vi "Range-check-csm-works.vi"(7 "UUID":string="Range check") -> ()   [LabVIEW 2018]
uses:
  <userlib>/_NEVSTOP/Communicable State Machine(CSM)/_Support/Typedef/_CSM_MODE.ctl
  API.ctl
  c61bc4df-35aa-4b4d-b5cf-ea0051ca23be.vi
  0e4ee468-faba-4892-866f-7e2dcb46ee8c.vi
  <userlib>/_NEVSTOP/Communicable State Machine(CSM)/AdvanceAPI/CSM - Revert Arguments-Safe String.vi
  <userlib>/_NEVSTOP/Communicable State Machine(CSM)/_Shared/Trim Single-line Text.vi
  <userlib>/_NEVSTOP/Communicable State Machine(CSM)/AdvanceAPI/CSM - Make String Arguments Safe.vi
  <userlib>/_NEVSTOP/Communicable State Machine(CSM)/AdvanceAPI/CSM - Break Down Multiple States String.vi
  <userlib>/_NEVSTOP/Communicable State Machine(CSM)/AdvanceAPI/CSM - Compact Multiple States.vi
  <userlib>/_NEVSTOP/Communicable State Machine(CSM)/AdvanceAPI/CSM - Keywords.vi
  <userlib>/_NEVSTOP/Communicable State Machine(CSM)/addons/API-String-Arugments-Support/_Support/Convert API String Arguments to Data(variant).vi
  <userlib>/_NEVSTOP/Communicable State Machine(CSM)/addons/API-String-Arugments-Support/_Support/Data To API String Arguments.vi
  <userlib>/_NEVSTOP/Communicable State Machine(CSM)/_Polymophic/Build Asynchronous Message with Arguments.vi
  <vilib>/regexp/Match Regular Expression.xnode
  <userlib>/_NEVSTOP/Communicable State Machine(CSM)/Communicable State Machine.lvlib
  <userlib>/_NEVSTOP/Communicable State Machine(CSM)/addons/Loop-Support/CSM Loop Support.lvlib
panel:
  out "输出簇":T2(array[cluster])
  out "Error Occurred":errorcluster
  out "State History":string
  # "借用CSM的works模式\n需要Timer CSM Works库---\n注意，由于退出机制的设置，本VI无论有多少个，一旦一个退出，其附带的所有的Timer-works都会退出\n没有办法，我并不能知道那个正在使用中\\\n本VI的API只能使用异步消息\n结果的返回是通过广播，所以需要你去注册对应广播"
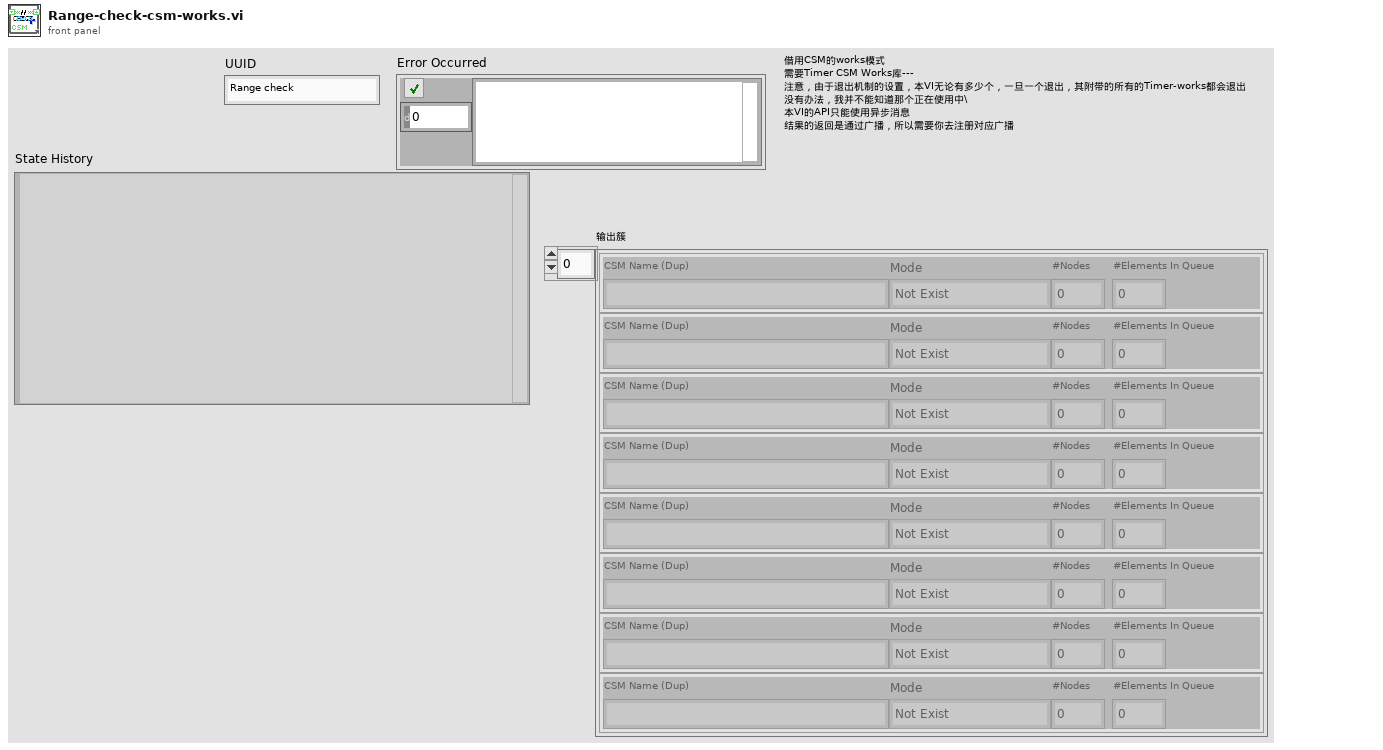
[diagram p1: front panel]
types:
  T1 = typedef "Communicable State Machine.lvlib/_CSM_MODE.ctl" = enum16{"Not Exist", "Stand Alone", "CSM", "Worker", "Worker Agent", "Chain Node", "Chain"}
  T2 = cluster{"CSM Name (Dup)":string, "Mode":T1, "#Nodes":i32, "#Elements In Queue":i32}[]
  T3 = enum32{"Invalid", "Standard", "Closed", "Hidden", "Minimized", "Maximized"}
  T4 = enum32{"invalid app kind", "Development System", "Run Time System", "Student Edition", "Embedded LabVIEW", "Evaluation", "Custom"}
  T5 = typedef "Communicable State Machine.lvlib/_CSM_Response Source Message.ctl" = cluster{"‘State":string, "’Arguments":string, "’Error":errorcluster}
  T6 = cluster{"Current VI Reference":refnum<vi>, "Close Panel on Exit?":bool}
  T7 = typedef "API.ctl" = cluster{"设定值上限":dbl, "设定值下限":dbl, "设定时间ms":u32, "超时时间ms":u32}
  T8 = cluster{"Core":cluster{"Current VI Reference":refnum<vi>, "Close Panel on Exit?":bool}, "Timing Parameters":T7, "Start":u32, "Esplase time":u32, "Success？":bool, "Time out？":bool, "Source":string, "ALL time":u32, "ALL Start":u32, "My name":string}
  T9 = cluster{"设定值上限":dbl, "设定值下限":dbl, "设定时间ms":dbl, "超时时间ms":dbl}
  T10 = cluster{"CSM Name (Dup)":string, "Mode":T1, "#Nodes":i32, "#Elements In Queue":i32}
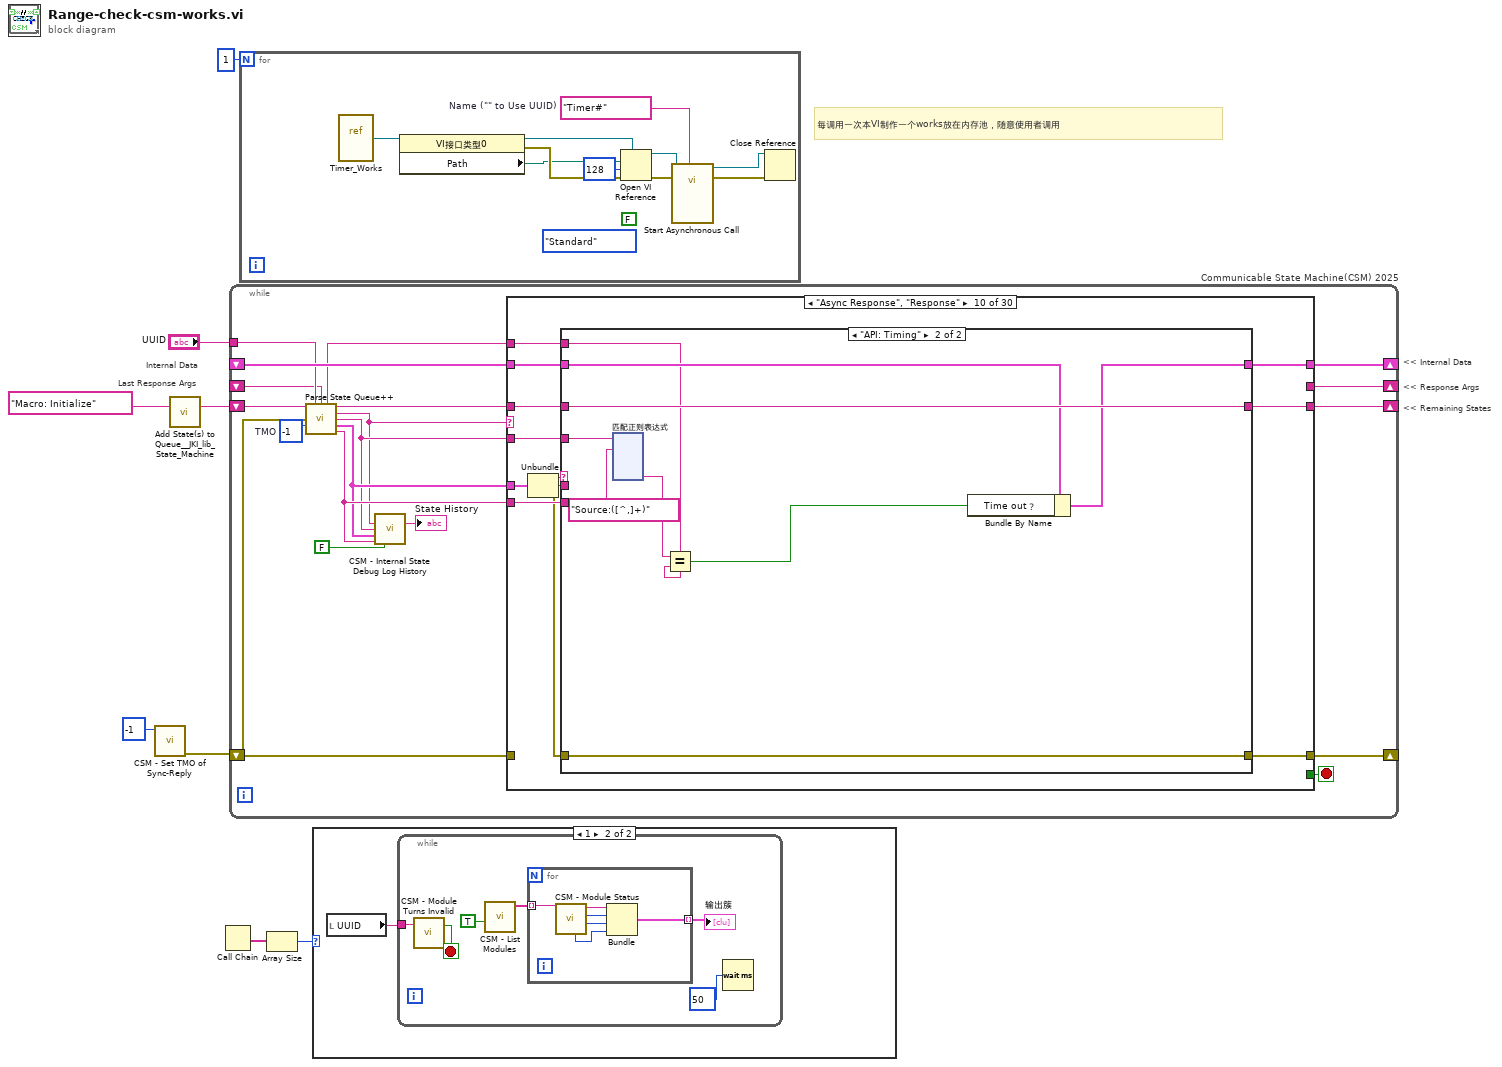
[diagram p0: block diagram]
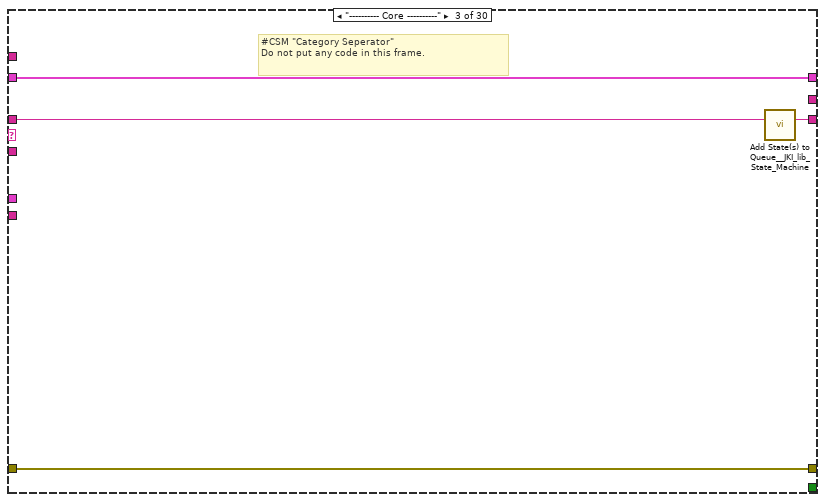
[diagram p5: hidden frame]
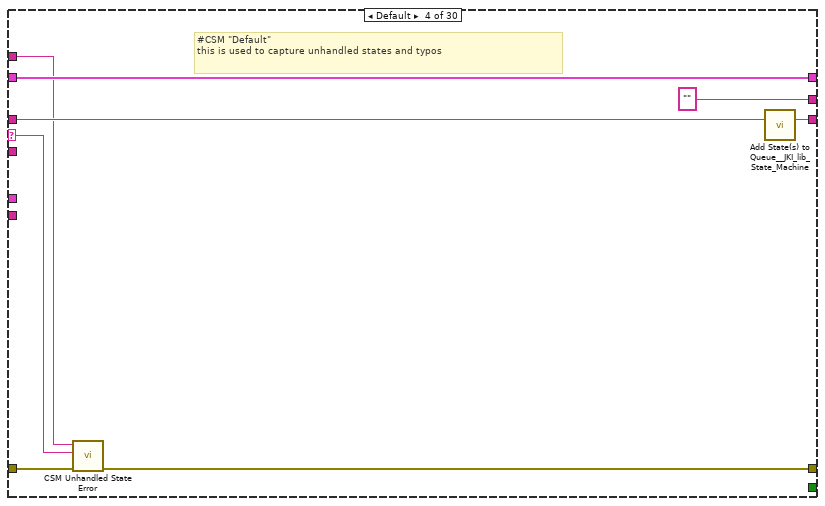
[diagram p6: hidden frame]
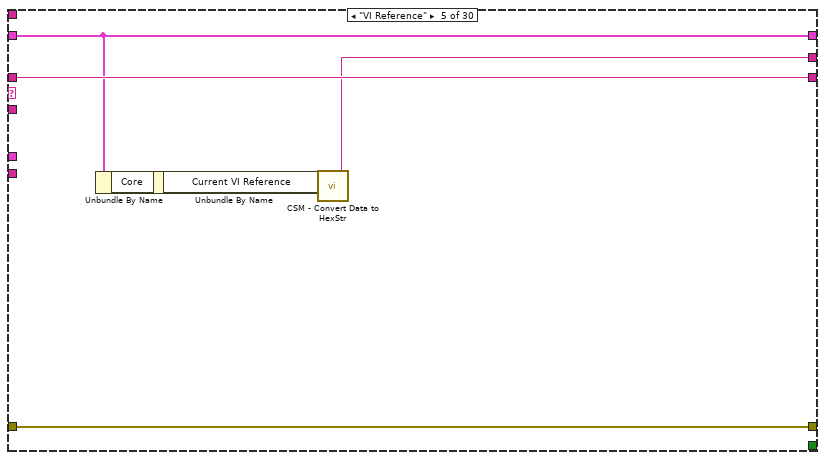
[diagram p7: hidden frame]
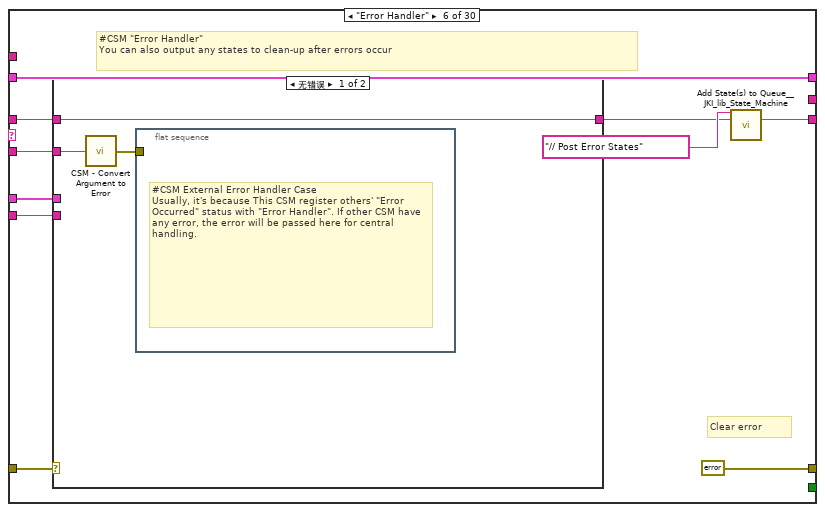
[diagram p8: hidden frame]
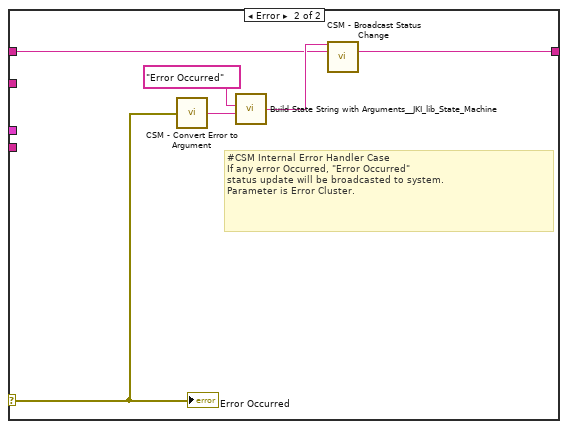
[diagram p9: hidden frame]
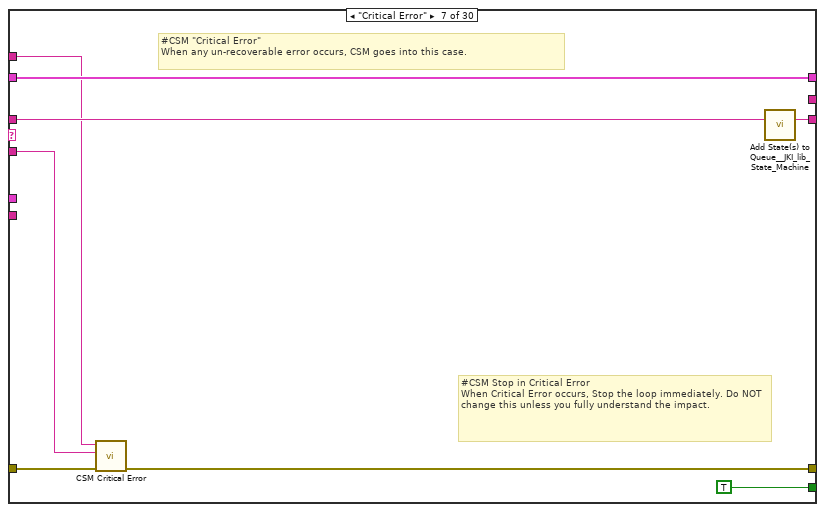
[diagram p10: hidden frame]
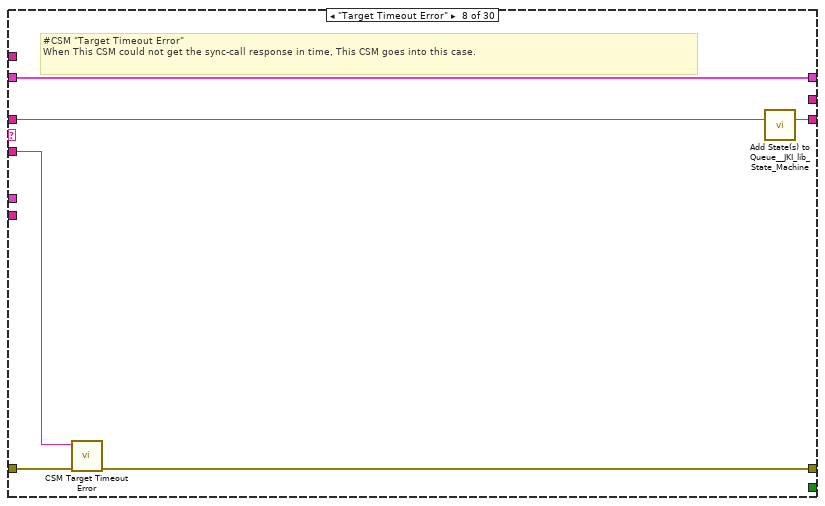
[diagram p11: hidden frame]
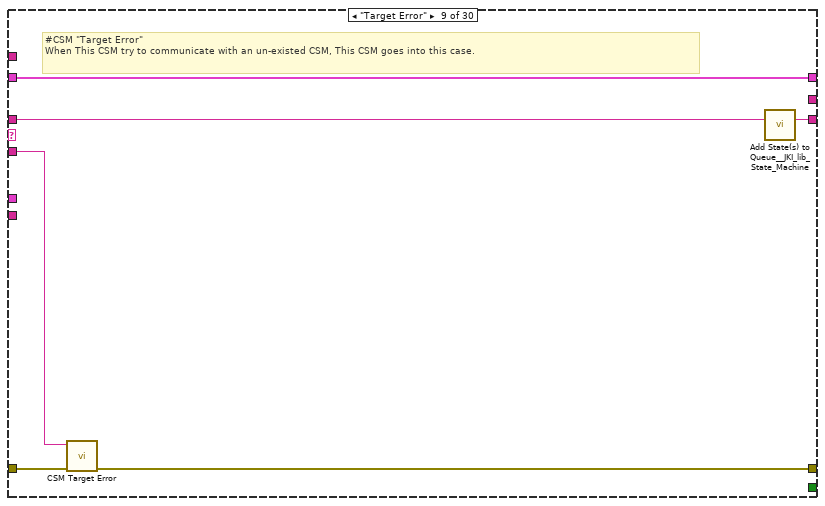
[diagram p12: hidden frame]
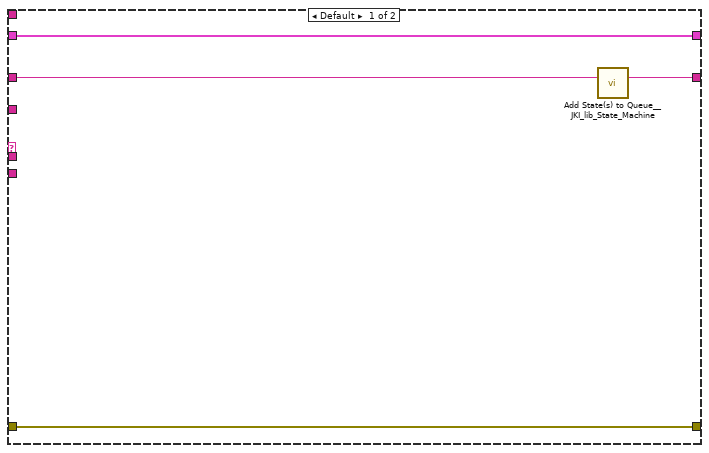
[diagram p13: hidden frame]
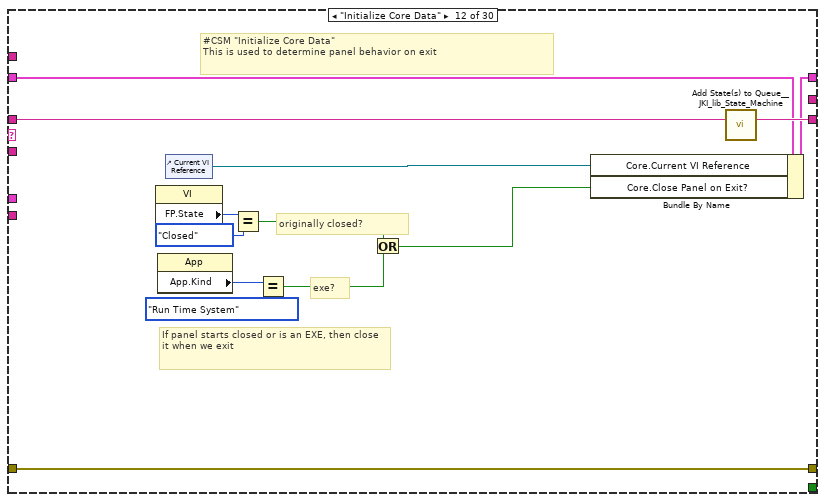
[diagram p15: hidden frame]
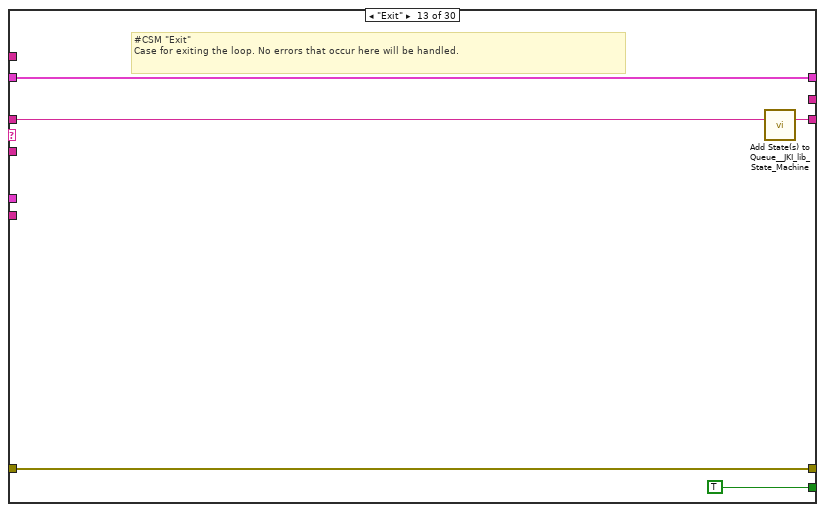
[diagram p16: hidden frame]
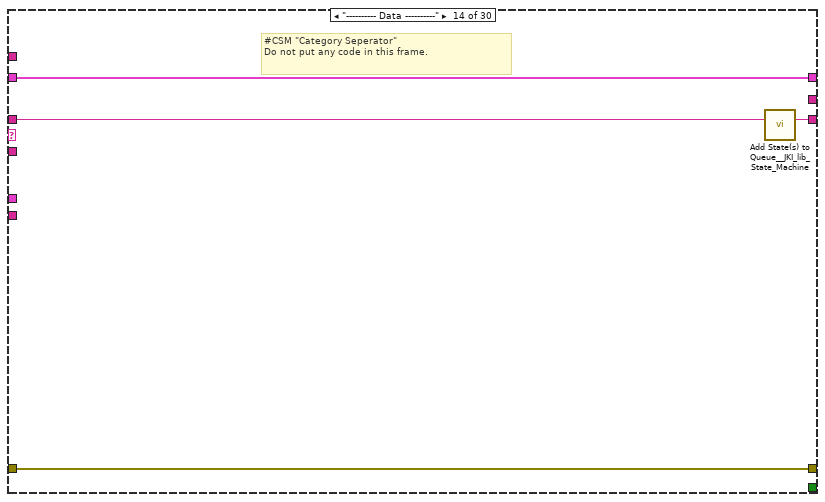
[diagram p17: hidden frame]
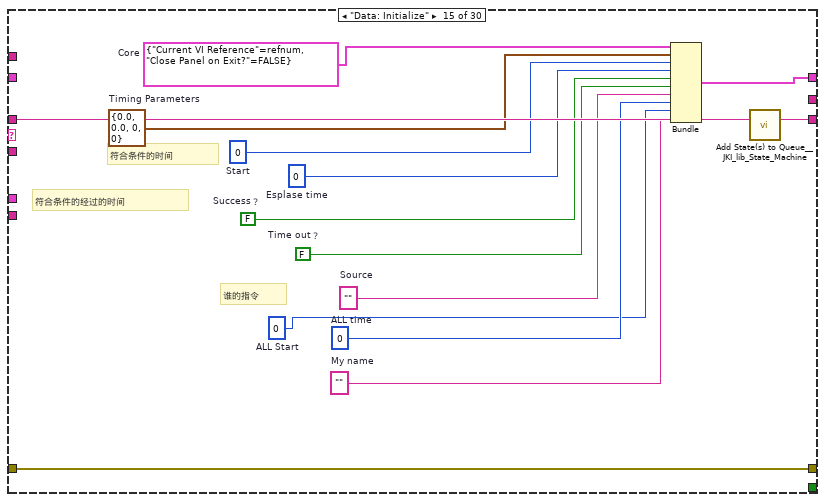
[diagram p18: hidden frame]
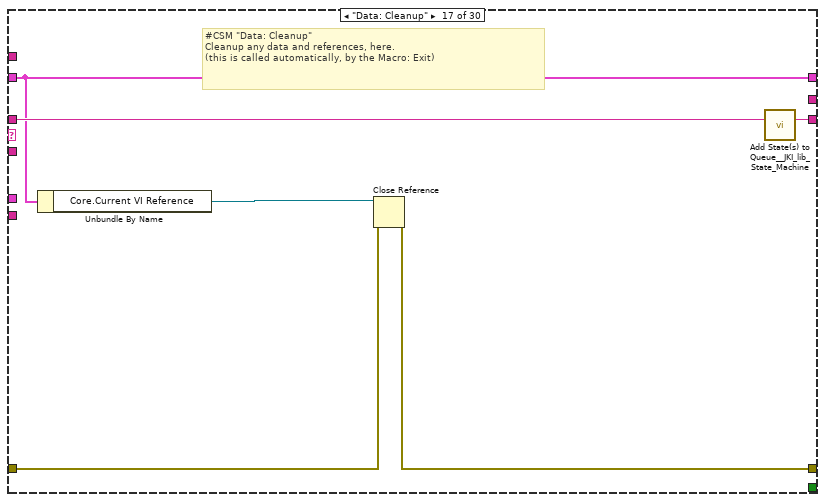
[diagram p20: hidden frame]
diagram:
  # "每调用一次本VI制作一个works放在内存池，随意使用者调用"
  # "Last Response Args"
  # "Internal Data"
  # "<< Internal Data"
  # "<< Response Args"
  # "<< Remaining States"
  n1 = call <userlib>:"CSM - Set TMO of Sync-Reply.vi"("TMO For Sync-Rep (ms) In"=-1) -> ("error out"=w3:errorcluster)  [unwired: 9 in, 1 out]
  n2 = call <vilib>:"Add State(s) to Queue__JKI_lib_State_Machine.vi"("State(s) in (\"\")"="Macro: Initialize" ("Init State(\"Macro: Initialize\")")) -> ("States Out"=w6:string)  [unwired: 14 in]
  n3 = Call Chain() -> (call chain=w1:string[])
  n4 = while "Communicable State Machine(CSM) 2025" {
    shift-right: [w22] -> _
    shift-left: _ -> [w21]
    shift-right: [w25] -> _
    shift-left: w3 -> [w11]
    shift-right: [w24] -> _
    shift-left: w6 -> [w26]
    tunnel: "UUID" -> [w18]
    shift-right: [w19] -> _
    shift-left: _ -> [w13]
    stop <- w23 stop-if-true
    w20 = -1  # TMO
    n5 = call <userlib>:"Parse State Queue++.vi"("State Queue"=w26, "Name (\"\" to Use UUID)"=w18, "Response Arguments"=w13, "Previous Error"=w11, "Dequeue (1 ms)"=w20) -> ("Name Used"=w12:string, "Remaining States"=w27:string, "Current State"=w14:string, "Arguments"=w15:string, "Additional Information"=w16:T5, "Source CSM"=w17:string)  [unwired: 5 in]
    n6 = call <userlib>:"CSM - Internal State Debug Log History.vi"("State"=w14, "Arguments (\"\")"=w15, ">> Response Source Message >>"=w16, "Source (\"\")"=w17, "Enable Periodic State Filter? (T)"=FALSE) -> ("Debug Log"=→"State History":string)  [unwired: 10 in]
    n7 = case shown="\"Async Response\", \"Response\"" w14 {
      selector: w14 -> [_ _ _ w41 _ _ _ _ _ _ _ _ _ _ _ _ _ _ _ _ _ _ _ _ _ _ _ _ w386 _]
      tunnel: w27 -> [w29 w33 w37 w45 w50 w55 w78 w84 w90 w101 w234 w247 w252 w256 w270 w273 w279 w283 w288 w294 w302 w305 w308 w320 w329 w338 w355 w378 w387 w393]
      tunnel: w15 -> [_ _ _ _ _ w54 w74 w81 w87 w96 _ _ _ _ _ _ _ _ _ _ _ _ w315 _ _ _ _ _ _ _]
      tunnel: w21 -> [w30 w32 w35 w43 w49 w60 w76 w82 w88 w92 w233 w241 w250 w254 _ w272 w274 w281 w286 w292 w300 w304 w316 w318 w327 w331 w354 w374 w385 w391]
      tunnel: [w28 w31 w34 w38 w51 errorcluster {"status"=FALSE, "code"=0, "source"=""} ("error out") w71 w79 w85 w102 w232 w235 w248 w253 w266 w271 w275 w280 w284 w290 w297 w303 w313 w317 w326 w336 w357 w376 w388 w390] -> w25
      tunnel: w11 -> [w28 w31 w34 w39 w51 w58 w72 w80 w86 _ w232 w235 w248 w253 w266 w271 w276 w280 w284 w290 w297 w303 w312 w317 w326 w336 w357 w376 w388 w390]
      tunnel: [w29 w33 w36 w44 w50 w56 w77 w83 w89 w100 w234 w246 w251 w255 w269 w273 w278 w282 w287 w293 w301 w305 w309 w319 w328 w337 w356 w377 w389 w392] -> w24
      tunnel: [_ _ _ _ _ _ TRUE _ _ _ _ _ TRUE _ _ _ _ _ _ _ _ _ _ _ _ _ _ _ _ _] -> w23
      tunnel: [w30 w32 w35 w43 w49 w60 w76 w82 w88 w99 w233 w245 w250 w254 w268 w272 w274 w281 w286 w292 w300 w304 w311 w318 w325 w331 w351 w374 w385 w391] -> w22
      tunnel: w17 -> [_ _ _ _ _ w53 _ _ _ w97 _ _ _ _ _ _ _ _ _ _ _ _ w306 _ _ _ _ _ _ _]
      tunnel: w16 -> [_ _ _ _ _ w52 _ _ _ w98 _ _ _ _ _ _ _ _ _ _ _ _ _ _ _ _ _ _ _ _]
      tunnel: [_ _ _ "" w46 _ _ _ _ _ _ _ _ _ _ _ _ _ _ _ _ _ _ _ _ _ _ _ _ _] -> w19
      tunnel: w12 -> [_ _ _ w40 _ _ w73 _ _ w91 _ _ _ _ _ _ _ _ _ _ _ _ _ _ _ _ _ _ _ _]
      frame "", "Idle" {
      }
      frame "CSM Documentation" {
      }
      frame "---------- Core ----------" {
        # "#CSM \"Category Seperator\"\nDo not put any code in this frame."
        n8 = call <vilib>:"Add State(s) to Queue__JKI_lib_State_Machine.vi"("State(s) in (\"\")"=w37) -> ("States Out"=w36:string)  [unwired: 14 in]
      }
      frame Default {
        # "#CSM \"Default\"\nthis is used to capture unhandled states and typos"
        n9 = call <userlib>:"CSM Unhandled State Error.vi"("error in (no error)"=w39, "Undefined State"=w41, "CSM Name"=w40) -> ("error out"=w38:errorcluster)  [unwired: 8 in]
        n10 = call <vilib>:"Add State(s) to Queue__JKI_lib_State_Machine.vi"("State(s) in (\"\")"=w45) -> ("States Out"=w44:string)  [unwired: 14 in]
      }
      frame "VI Reference" {
        n11 = Unbundle By Name(w49) -> ("Core"=w48:T6)
        n12 = Unbundle By Name(w48) -> ("Current VI Reference"=w47:refnum<vi>)
        n13 = call <userlib>:"CSM - Convert Data to HexStr.vi"("Variant"=w47) -> ("HEX String (0-9,A-F)"=w46:string)  [unwired: 8 in]
      }
      frame "Error Handler" {
        # "#CSM \"Error Handler\"\nYou can also output any states to clean-up after errors occur"
        # "Clear error"
        n14 = case shown="无错误" w58 {
          selector: w58 -> [_ w65]
          tunnel: [w64 w67] -> w57
          tunnel: w55 -> [w64 w66]
          tunnel: w54 -> [w63 _]
          tunnel: w53 -> [_ _]
          tunnel: w52 -> [_ _]
          frame No Error {
            n15 = call <userlib>:"CSM - Convert Argument to Error.vi"("Argument"=w63) -> ("Error"=w62:errorcluster)  [unwired: 4 in]
            n16 = flat-sequence {
              tunnel: w62 -> [_]
              frame #0 {
                # "#CSM External Error Handler Case\nUsually, it's because This CSM register others' \"Error Occurred\" status with \"Error Handler\". If other CSM have any error, the error will be passed here for central handling."
              }
            }
          }
          frame Error {
            # "#CSM Internal Error Handler Case \nIf any error Occurred, \"Error Occurred\" \nstatus update will be broadcasted to system.\nParameter is Error Cluster."
            n17 = call <userlib>:"CSM - Convert Error to Argument.vi"("Error"=w65) -> ("Argument"=w69:string)  [unwired: 4 in]
            n18 = call <vilib>:"Build State String with Arguments__JKI_lib_State_Machine.vi"("Arguments (\"\")"=w69, "State"="Error Occurred" ("Status with Arguments")) -> ("State with Arguments"=w68:string)  [unwired: 4 in]
            n19 = call <userlib>:"CSM - Broadcast Status Change.vi"("Status With Arguments"=w68, "State Queue"=w66) -> ("Remaining States"=w67:string)  [unwired: 13 in]
            "Error Occurred" <- w65
          }
        }
        n20 = call <vilib>:"Add State(s) to Queue__JKI_lib_State_Machine.vi"("State(s) in Front (\"\")"="// Post Error States", "State(s) in (\"\")"=w57) -> ("States Out"=w56:string)  [unwired: 13 in]
      }
      frame "Critical Error" {
        # "#CSM \"Critical Error\"\nWhen any un-recoverable error occurs, CSM goes into this case."
        # "#CSM Stop in Critical Error\nWhen Critical Error occurs, Stop the loop immediately. Do NOT change this unless you fully understand the impact."
        n21 = call <userlib>:"CSM Critical Error.vi"("error in (no error)"=w72, "Arugments (As Reason)"=w74, "CSM Name"=w73) -> ("error out"=w71:errorcluster)  [unwired: 8 in]
        n22 = call <vilib>:"Add State(s) to Queue__JKI_lib_State_Machine.vi"("State(s) in (\"\")"=w78) -> ("States Out"=w77:string)  [unwired: 14 in]
      }
      frame "Target Timeout Error" {
        # "#CSM \"Target Timeout Error\"\nWhen This CSM could not get the sync-call response in time, This CSM goes into this case."
        n23 = call <userlib>:"CSM Target Timeout Error.vi"("error in (no error)"=w80, "Arguments (As CSM Name)"=w81) -> ("error out"=w79:errorcluster)  [unwired: 9 in]
        n24 = call <vilib>:"Add State(s) to Queue__JKI_lib_State_Machine.vi"("State(s) in (\"\")"=w84) -> ("States Out"=w83:string)  [unwired: 14 in]
      }
      frame "Target Error" {
        # "#CSM \"Target Error\"\nWhen This CSM try to communicate with an un-existed CSM, This CSM goes into this case."
        n25 = call <userlib>:"CSM Target Error.vi"("error in (no error)"=w86, "Arguments (As CSM Name)"=w87) -> ("error out"=w85:errorcluster)  [unwired: 9 in]
        n26 = call <vilib>:"Add State(s) to Queue__JKI_lib_State_Machine.vi"("State(s) in (\"\")"=w90) -> ("States Out"=w89:string)  [unwired: 14 in]
      }
      frame "Async Response", "Response" {
        n27 = Unbundle(w98) -> ("‘State"=w95:string, "’Arguments"=w94:string, "’Error"=w93:errorcluster)
        n28 = case shown="\"API: Timing\"" w95 {
          tunnel: [w104 w115] -> w100
          tunnel: w101 -> [w105 w115]
          tunnel: [w103 w110] -> w99
          tunnel: [w106 w114] -> w102
          tunnel: w93 -> [w106 w114]
          tunnel: w97 -> [_ _]
          tunnel: w96 -> [_ w113]
          tunnel: w94 -> [_ _]
          tunnel: w92 -> [w103 w108]
          tunnel: w91 -> [_ w107]
          frame Default {
            n29 = call <vilib>:"Add State(s) to Queue__JKI_lib_State_Machine.vi"("State(s) in (\"\")"=w105) -> ("States Out"=w104:string)  [unwired: 14 in]
          }
          frame "API: Timing" {
            n30 = xnode "匹配正则表达式"("输入字符串"=w113, "正则表达式"="Source:([^,]+)") -> ("子匹配 1"=w111:string)  [unwired: 4 in, 5 out]
            n31 = Equal?(x=w111, y=w107) -> (x = y?=w109:bool)
            n32 = Bundle By Name(cluster=w108, "Time out？"=w109) -> (w110:T8)
          }
        }
      }
      frame "Async Message Posted" {
        # "#CSM \"Async Message Posted\"\nAfter Async Message is posted (-> or ->| ), CSM goes to this state for post-action.\nYou can use Argument - State to tell which Async Message is called."
      }
      frame "Initialize Core Data" {
        # "#CSM \"Initialize Core Data\"\nThis is used to determine panel behavior on exit"
        # "originally closed?"
        # "exe?"
        # "If panel starts closed or is an EXE, then close it when we exit"
        n33 = property class="VI"() -> ("FP.State"=w238:T3)  [unwired: 2 in, 2 out]
        n34 = property class="App"() -> ("App.Kind"=w244:T4)  [unwired: 2 in, 2 out]
        n35 = control-ref of="Current VI Reference"() -> (w239:refnum<vi>)
        n36 = Equal?(x=w238, y=T3."Closed" ("Front Panel Window:State")) -> (x = y?=w236:bool)
        n37 = Equal?(x=w244, y=T4."Run Time System" ("Application:Kind")) -> (x = y?=w242:bool)
        n38 = Or(x=w236, y=w242) -> (x .or. y?=w240:bool)
        n39 = Bundle By Name(cluster=w241, "Core.Current VI Reference"=w239, "Core.Close Panel on Exit?"=w240) -> (w245:T8)
        n40 = call <vilib>:"Add State(s) to Queue__JKI_lib_State_Machine.vi"("State(s) in (\"\")"=w247) -> ("States Out"=w246:string)  [unwired: 14 in]
      }
      frame "Exit" {
        # "#CSM \"Exit\"\nCase for exiting the loop. No errors that occur here will be handled."
        n41 = call <vilib>:"Add State(s) to Queue__JKI_lib_State_Machine.vi"("State(s) in (\"\")"=w252) -> ("States Out"=w251:string)  [unwired: 14 in]
      }
      frame "---------- Data ----------" {
        # "#CSM \"Category Seperator\"\nDo not put any code in this frame."
        n42 = call <vilib>:"Add State(s) to Queue__JKI_lib_State_Machine.vi"("State(s) in (\"\")"=w256) -> ("States Out"=w255:string)  [unwired: 14 in]
      }
      frame "Data: Initialize" {
        w257 = ""  # My name
        w258 = u32 0  # ALL Start
        w259 = u32 0  # ALL time
        w260 = ""  # Source
        w261 = FALSE  # Time out？
        w262 = u32 0  # Start
        w263 = u32 0  # Esplase time
        w264 = FALSE  # Success？
        w265 = T7 {"设定值上限"=0.0, "设定值下限"=0.0, "设定时间ms"=0, "超时时间ms"=0}  # Timing Parameters
        w267 = T6 {"Current VI Reference"=refnum, "Close Panel on Exit?"=FALSE}  # Core
        # "谁的指令"
        # "符合条件的经过的时间"
        # "符合条件的时间"
        n43 = Bundle("Core"=w267, "Timing Parameters"=w265, "Start"=w262, "Esplase time"=w263, "Success？"=w264, "Time out？"=w261, "Source"=w260, "ALL time"=w259, "ALL Start"=w258, "My name"=w257) -> (w268:T8)  [unwired: 1 in]
        n44 = call <vilib>:"Add State(s) to Queue__JKI_lib_State_Machine.vi"("State(s) in (\"\")"=w270) -> ("States Out"=w269:string)  [unwired: 14 in]
      }
      frame "Data: Update Indicators" {
      }
      frame "Data: Cleanup" {
        # "#CSM \"Data: Cleanup\"\nCleanup any data and references, here.\n(this is called automatically, by the Macro: Exit)"
        n45 = Unbundle By Name(w274) -> ("Core.Current VI Reference"=w277:refnum<vi>)
        n46 = Close Reference(reference=w277, error in (no error)=w276) -> (error out=w275:errorcluster)
        n47 = call <vilib>:"Add State(s) to Queue__JKI_lib_State_Machine.vi"("State(s) in (\"\")"=w279) -> ("States Out"=w278:string)  [unwired: 14 in]
      }
      frame "---------- Macro ----------" {
        # "#CSM \"Category Seperator\"\nDo not put any code in this frame."
        n48 = call <vilib>:"Add State(s) to Queue__JKI_lib_State_Machine.vi"("State(s) in (\"\")"=w283) -> ("States Out"=w282:string)  [unwired: 14 in]
      }
      frame "Macro: Initialize" {
        # "#CSM \"Macro: Initialize\"\nInitialization Macro (This is called once, when the VI starts)"
        n49 = call <vilib>:"Add State(s) to Queue__JKI_lib_State_Machine.vi"("State(s) in Front (\"\")"="Data: Initialize\nInitialize Core Data\nData: Update Indicators\n", "State(s) in (\"\")"=w288) -> ("States Out"=w287:string)  [unwired: 13 in]
      }
      frame "Macro: Range check" {
        # "由于这个优先级\n问题会导致信息\n的回复出现问题，\n所以我直接让他不\n返回，结束了就\n广播"
        # "#CSM \"Macro: Initialize\"\nInitialization Macro (This is called once, when the VI starts)"
        n50 = call <userlib>:"CSMLS - Define Loop State(s).vi"("Loop States"="Action: Initialize\nAction: Start\nAction: check\nAction: Loop check-><Loop>\nAction: Stop\n", "States Queue"=w294, "Add to Front? (F)"=FALSE) -> ("Remaining States"=w293:string)  [unwired: 12 in]
      }
      frame "Macro: Exit" {
        # "#CSM \"Macro: Exit\"\nExit Macro (This is called once, when the VI exits)"
        n51 = call <userlib>:"CSM - Build Exit Messages of CSMs.vi"("CSMs"=string[] ["Timer"]) -> ("States"=w295:string)  [unwired: 14 in]
        n52 = call <vilib>:"Add State(s) to Queue__JKI_lib_State_Machine.vi"("State(s) in Front (\"\")"=w295, "State(s) at Back (\"\")"="Data: Cleanup\nExit") -> ("States Out"=w298:string)  [unwired: 13 in]
        n53 = call <vilib>:"Add State(s) to Queue__JKI_lib_State_Machine.vi"("State(s) in Front (\"\")"=w298, "State(s) in (\"\")"=w302) -> ("States Out"=w301:string)  [unwired: 13 in]
      }
      frame "---------- API ----------" {
        # "#CSM \"Category Seperator\"\nDo not put any code in this frame."
      }
      frame "API: Range check" {
        w314 = T9 {"设定值上限"=0.0, "设定值下限"=0.0, "设定时间ms"=0.0, "超时时间ms"=0.0}  # Timing Parameters
        n54 = call "Convert API String Arguments to Data.vim"("Reference Type"=w314, "error in (no error)"=w312, "API String"=w315) -> ("error out"=w313:errorcluster, "Data"=w310:T9)  [unwired: 5 in]
        n55 = Bundle By Name(cluster=w316, "Timing Parameters"=w310, "Source"=w306) -> (w311:T8)
        n56 = call <vilib>:"Add State(s) to Queue__JKI_lib_State_Machine.vi"("State(s) in Front (\"\")"="Macro: Range check" ("State(s) in Front (\"\")"), "State(s) in (\"\")"=w308) -> ("States Out"=w309:string)  [unwired: 13 in]
      }
      frame "---------- Action ----------" {
        # "#CSM \"Category Seperator\"\nDo not put any code in this frame."
        n57 = call <vilib>:"Add State(s) to Queue__JKI_lib_State_Machine.vi"("State(s) in (\"\")"=w320) -> ("States Out"=w319:string)  [unwired: 14 in]
      }
      frame "Action: Initialize" {
        w324 = FALSE ("Success？")
        # "#CSM \"Internal State\"\nThis category is used for holding internal states"
        n58 = Tick Count (ms)() -> (millisecond timer value=w322:u32)
        n59 = Bundle By Name(cluster=w327, "Start"=w322, "Esplase time"=0 ("Start"), "Success？"=w324, "Time out？"=w324, "ALL Start"=w322, "ALL time"=u32 0) -> (w325:T8)
        n60 = call <vilib>:"Add State(s) to Queue__JKI_lib_State_Machine.vi"("State(s) in (\"\")"=w329) -> ("States Out"=w328:string)  [unwired: 14 in]
      }
      frame "Action: Start" {
        # "给倒计时先做上"
        n61 = Unbundle By Name(w331) -> ("Timing Parameters.超时时间ms"=w330:u32)
        n62 = call "Convert Data To API String Arguments.vim"("Data"=w330) -> ("API String"=w333:string)  [unwired: 7 in, 1 out]
        n63 = call-poly <userlib>:"Build Message with Arguments++.vi"("State With Arguments"="API: Timing", "Arguments (\"\")"=w333, "Target Module (\"\")"="Timer" ("Target Module (\"\")")) -> ("CSM Message String"=w332:string)  [unwired: 12 in]
        n64 = call <vilib>:"Add State(s) to Queue__JKI_lib_State_Machine.vi"("State(s) in Front (\"\")"=w332, "State(s) in (\"\")"=w338) -> ("States Out"=w337:string)  [unwired: 13 in]
      }
      frame "Action: check" {
        n65 = Unbundle By Name(w354) -> ("Timing Parameters.设定值上限"=w353:dbl, "Timing Parameters.设定值下限"=w352:dbl, "Timing Parameters.设定时间ms"=w348:u32, "Esplase time"=w346:u32, "Start"=w344:u32, "ALL Start"=w341:u32)
        n66 = Wait (ms)(milliseconds to wait=u32 1 ("等待时间（毫秒）")) -> ()  [unwired: 1 out]
        n67 = Tick Count (ms)() -> (millisecond timer value=w340:u32)
        n68 = In Range and Coerce(upper limit=w353, x=0.0, lower limit=w352) -> (In Range?=w349:bool)  [unwired: 1 out]
        n69 = case shown="真" w349 {
          tunnel: [0 w361] -> w339
          tunnel: [w358 w362] -> w345
          tunnel: w344 -> [_ w362]
          tunnel: w340 -> [w358 w360]
          frame False {
          }
          frame True {
            n70 = Subtract(x=w360, y=w362) -> (x-y=w361:u32)
          }
        }
        n71 = Less Or Equal?(x=w348, y=w346) -> (x <= y?=w347:bool)
        n72 = Subtract(x=w340, y=w341) -> (x-y=w342:u32)
        n73 = Bundle By Name(cluster=w354, "Success？"=w347, "Start"=w345, "Esplase time"=w339, "ALL time"=w342) -> (w351:T8)
        n74 = call <vilib>:"Add State(s) to Queue__JKI_lib_State_Machine.vi"("State(s) in (\"\")"=w355) -> ("States Out"=w356:string)  [unwired: 14 in]
      }
      frame "Action: Stop" {
        n75 = Unbundle By Name(w374) -> ("Source"=w373:string, "Time out？"=w372:bool, "Success？"=w371:bool, "Esplase time"=w368:u32, "ALL time"=w367:u32)
        n76 = Boolean To (0,1)(Boolean=w372) -> (0, 1=w370:i16)
        n77 = Boolean To (0,1)(Boolean=w371) -> (0, 1=w369:i16)
        n78 = Format Into String(format string="Source:%s,Time out:%d,Success:%d,Esplase time:%d,All time:%d" ("格式字符串"), w373, w370, w369, w368, w367) -> (resulting string=w363:string)  [unwired: 2 in, 1 out]
        n79 = Format Into String(format string="%s" ("格式字符串"), initial string="Range Check Completd>>" ("State With Arguments"), w363) -> (resulting string=w366:string)  [unwired: 1 in, 1 out]
        n80 = call <userlib>:"CSM - Broadcast Status Change.vi"("Status With Arguments"=w366, "State Queue"=w378) -> ("Remaining States"=w377:string)  [unwired: 13 in]
      }
      frame "Action: Loop check" {
        # "#CSM \"Internal State\"\nThis category is used for holding internal states"
        n81 = Unbundle By Name(w385) -> ("Time out？"=w379:bool, "Success？"=w384:bool)
        n82 = Or(x=w379, y=w384) -> (x .or. y?=w380:bool)
        n83 = Select(t="Action: Loop quit", s=w380, f="Action: check") -> (s? t:f=w381:string)
        n84 = call <userlib>:"CSMLS - Append Continuous State.vi"("Loop State(s) And Arguments"=w381, "Continous State"=w386, "States Queue"=w387) -> ("Remaining States"=w389:string)  [unwired: 8 in]
      }
      frame "Action: Loop quit" {
        # "#CSM \"Internal State\"\nThis category is used for holding internal states"
        n85 = call <userlib>:"CSMLS - Remove Loop Tag and previous State(s) to Break.vi"("States Queue"=w393) -> ("Remaining States"=w392:string)  [unwired: 10 in]
      }
    }
  }
  n86 = for {
    N: 1 -> [_]
    (unwired) T3."Standard" ("状态")
    (unwired) FALSE ("激活？")
    w402 = "Timer#"  # Name ("" to Use UUID)
    n87 = vi-ref "Timer_Works.vi"() -> (w397:refnum<vi>)
    n88 = property class="VI接口类型0"(reference=w397) -> (reference out=w401:refnum<vi>, error out=w399:errorcluster, "Path"=w398:path)  [unwired: 1 in]
    n89 = Open VI Reference(type specifier VI Refnum (for type only)=w401, vi path=w398, options=128, error in (no error)=w399) -> (vi reference=w400:refnum<vi>, error out=w396:errorcluster)  [unwired: 2 in]
    n90 = call-by-ref "Start Asynchronous Call"(reference=w400, error in=w396, "Name(\"\" to use uuid)"=w402) -> (reference out=w395:refnum<vi>, error out=w394:errorcluster)  [unwired: 11 in]
    n91 = Close Reference(reference=w395, error in (no error)=w394) -> ()  [unwired: 1 out]
  }
  n92 = Array Size(array=w1) -> (size(s)=w2:i32)
  n93 = case shown="1" w2 {
    frame 0, Default {
    }
    frame 1 {
      n94 = local read "UUID"() -> (w404:string)
      n95 = while {
        tunnel: w404 -> [w407]
        stop <- w406 stop-if-true
        n96 = call <userlib>:"CSM - Module Turns Invalid.vi"("CSM Name"=w407) -> ("Turn Invalid (Exit)?"=w406:bool)  [unwired: 2 in]
        n97 = call <userlib>:"CSM - List Modules.vi"("With Nodes? (F)"=TRUE) -> ("Module Names"=w410:string[])  [unwired: 9 in, 1 out]
        n98 = for {
          tunnel: w410 -> [w416] mode=indexing
          tunnel: [w411] -> w409 mode=indexing
          n99 = call <userlib>:"CSM - Module Status.vi"("CSM Name"=w416) -> ("#Nodes"=w413:i32, "Mode"=w414:T1, "CSM Name (Dup)"=w415:string, "#Elements In Queue"=w412:i32)  [unwired: 6 in, 1 out]
          n100 = Bundle("CSM Name (Dup)"=w415, "Mode"=w414, "#Nodes"=w413, "#Elements In Queue"=w412) -> (w411:T10)  [unwired: 1 in]
        }
        "输出簇" <- w409
        n101 = Wait (ms)(milliseconds to wait=u32 50 ("等待时间（毫秒）")) -> ()  [unwired: 1 out]
      }
    }
  }
